vi "order-tracks-test.vi"(1 "Order Settings":T1={"pulses per rev"=1, "trigger level (V)"=2.5, "max order"=64.0, "order resolution"=0.1, "window"=1, "averaging parameters"={"averaging mode"=enum."No averaging", "weighting mode"=enum."Linear", "number of averages"=1, "linear mode"=enum."One shot"}, "order ranges"=[{"start"=0.8, "stop"=1.2}, {"start"=1.8, "stop"=2.2}, {"start"=23.8, "stop"=24.2}]}, 4 "Noise (g rms)":dbl=0.01, 5 "Phases (deg)":dbl[](array[numeric])=[30.0, 0.0, 0.0, 0.0, 0.0], 6 "Orders":dbl[](array[numeric])=[1.0, 2.0, 3.57, 4.0, 24.0], 7 "Amplitudes (g pk)":dbl[](array[numeric])=[0.5, 0.2, 0.1, 0.05, 0.3], 8 "error in (no error)":errorcluster, 9 "Duration (s)":dbl=30.0, 10 "Ramps":T2(array[cluster]), 11 "Base RPM":dbl=3000.0) -> (0 "error out":errorcluster, 2 "True RPM":dbl[](array[numeric]), 3 "Values":dbl[][](array[numeric]))   [LabVIEW 2026]
doc: "Unit-test harness for OrderTracks.vi. Synthesises accel (sum of order sines, peak amplitudes, uniform noise) and a 1 ppr 0-5 V square tach (rising edge at shaft angle 0) for rpm(t) = Base RPM + sum of linear ramps, cuts it into 0.1 s blocks (5120 S @ 51.2 kS/s) and calls OrderTracks.vi block by block like FlexLogger Process.vi does (Data In = [accel, tach], reset? TRUE on block 0). Returns NUMERIC arrays only: Values [blocks x (2 + order ranges)] = RPM, order amplitudes (g rms); True RPM at each block centre."
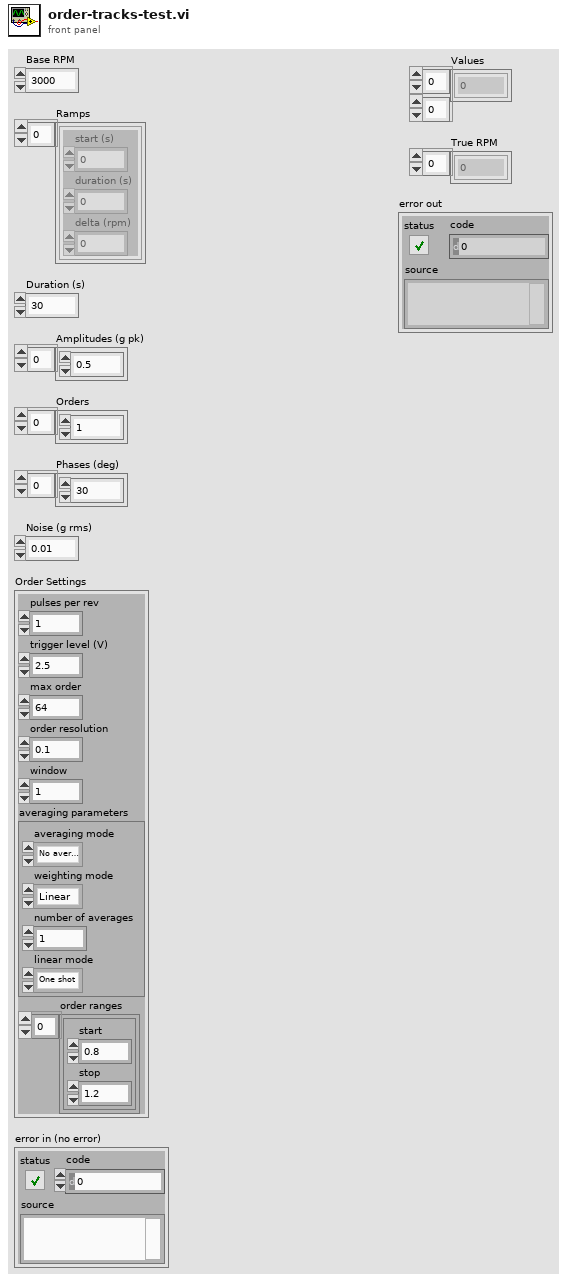
[diagram p1: front panel]
types:
  T1 = cluster{"pulses per rev":i32, "trigger level (V)":dbl, "max order":dbl, "order resolution":dbl, "window":u32, "averaging parameters":cluster{"averaging mode":enum16{"No averaging", "Vector averaging", "RMS averaging", "Peak hold"}, "weighting mode":enum16{"Linear", "Exponential"}, "number of averages":u32, "linear mode":enum16{"One shot", "Auto restart"}}, "order ranges":cluster{"start":dbl, "stop":dbl}[]}
  T2 = cluster{"start (s)":dbl, "duration (s)":dbl, "delta (rpm)":dbl}[]
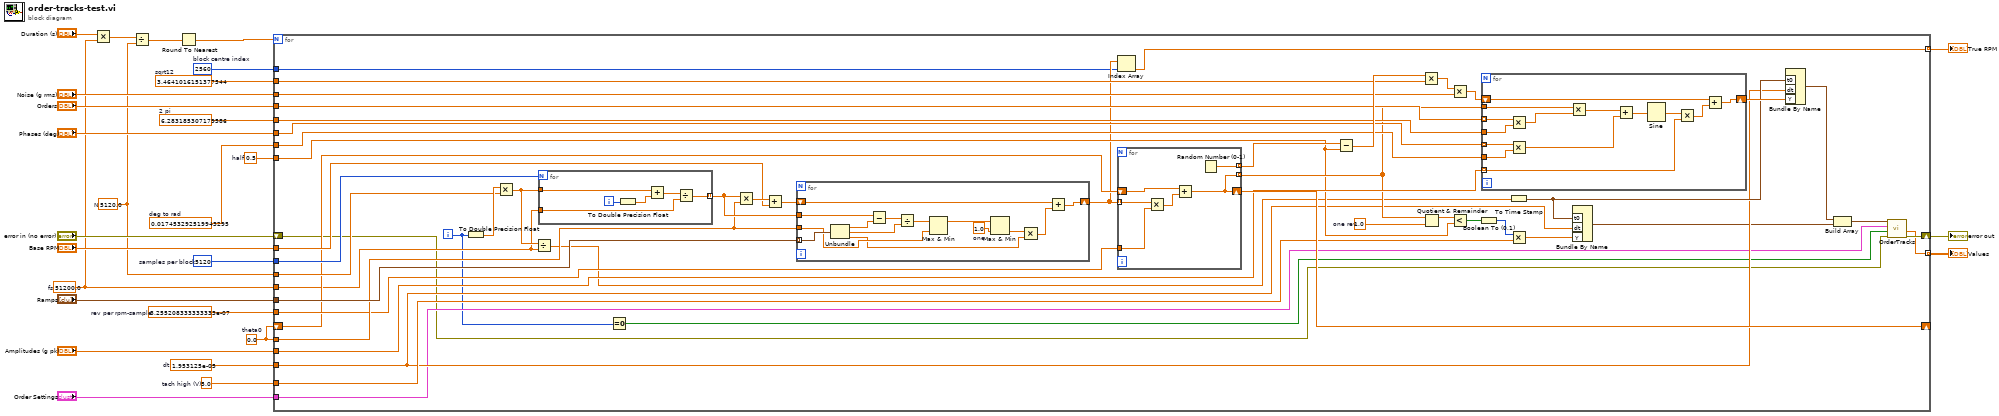
[diagram p0: block diagram]
diagram:
  w6 = 2560  # block centre index
  w7 = 5.0  # tach high (V)
  w8 = 6.283185307179586  # 2 pi
  w9 = 0.017453292519943295  # deg to rad
  w10 = 0.5  # half
  w11 = 3.4641016151377544  # sqrt12
  w12 = 1.953125e-05  # dt
  w13 = 3.255208333333333e-07  # rev per rpm-sample
  w5 = 0.0  # theta0
  w14 = 5120.0  # N
  w15 = 5120  # samples per block
  w16 = 51200.0  # fs
  n1 = Multiply(x="Duration (s)", y=w16) -> (x*y=w26:dbl)
  n2 = Divide(x=w26, y=w14) -> (x/y=w25:dbl)
  n3 = Round To Nearest(number=w25) -> (nearest integer value=w4:dbl)
  n4 = for {
    N: w4 -> [_]
    shift-right: [w66] -> _
    shift-left: w5 -> [w65]
    shift-right: [w33] -> w1
    shift-left: "error in (no error)" -> [w34]
    tunnel: "Base RPM" -> [w72]
    tunnel: "Ramps" -> [w71]
    tunnel: "Amplitudes (g pk)" -> [w58]
    tunnel: "Orders" -> [w59]
    tunnel: "Phases (deg)" -> [w57]
    tunnel: "Noise (g rms)" -> [w60]
    tunnel: "Order Settings" -> [w36]
    tunnel: w16 -> [w45]
    tunnel: w15 -> [w74]
    tunnel: w14 -> [w75]
    tunnel: w13 -> [w67]
    tunnel: w12 -> [w41]
    tunnel: w11 -> [w62]
    tunnel: w10 -> [w50]
    tunnel: w9 -> [w55]
    tunnel: w8 -> [w56]
    tunnel: w7 -> [w47]
    tunnel: w6 -> [w31]
    tunnel: w5 -> [w69]
    tunnel: [w30] -> w3 mode=indexing
    tunnel: [w29] -> w2 mode=indexing
    i -> [w28]
    w52 = 1.0  # one rev
    n5 = To Double Precision Float(number=w28) -> (double precision float=w76:dbl)
    n6 = Multiply(x=w76, y=w75) -> (x*y=w46:dbl)
    n7 = Divide(x=w46, y=w45) -> (x/y=w44:dbl)
    n8 = for {
      N: w74 -> [_]
      tunnel: w46 -> [w116]
      tunnel: w45 -> [w113]
      tunnel: [w112] -> w70 mode=indexing
      i -> [w111]
      n9 = To Double Precision Float(number=w111) -> (double precision float=w115:dbl)
      n10 = Add(x=w116, y=w115) -> (x+y=w114:dbl)
      n11 = Divide(x=w114, y=w113) -> (x/y=w112:dbl)
    }
    n12 = Equal To 0?(x=w28) -> (x = 0?=w35:bool)
    n13 = Multiply(x=w70, y=w69) -> (x*y=w73:dbl[])
    n14 = Add(x=w73, y=w72) -> (x+y=w68:dbl[])
    n15 = for {
      tunnel: w71 -> [w110] mode=indexing
      tunnel: w70 -> [w109]
      tunnel: w69 -> [w104]
      shift-right: [w97] -> w32
      shift-left: w68 -> [w99]
      w102 = 1.0  # one
      n16 = Unbundle(w110) -> ("start (s)"=w108:dbl, "duration (s)"=w106:dbl, "delta (rpm)"=w100:dbl)
      n17 = Subtract(x=w109, y=w108) -> (x-y=w107:dbl[])
      n18 = Divide(x=w107, y=w106) -> (x/y=w105:dbl[])
      n19 = Max & Min(x=w105, y=w104) -> (max(x,y)=w103:dbl[])  [unwired: 1 out]
      n20 = Max & Min(x=w103, y=w102) -> (min(x,y)=w101:dbl[])  [unwired: 1 out]
      n21 = Multiply(x=w101, y=w100) -> (x*y=w98:dbl[])
      n22 = Add(x=w99, y=w98) -> (x+y=w97:dbl[])
    }
    n23 = Index Array(array=w32, index=w31) -> (element=w29:dbl)
    n24 = for {
      tunnel: w32 -> [w96] mode=indexing
      tunnel: w67 -> [w95]
      shift-right: [w92] -> w66
      shift-left: w65 -> [w94]
      tunnel: [w92] -> w53 mode=indexing
      tunnel: [w91] -> w64 mode=indexing
      n25 = Multiply(x=w96, y=w95) -> (x*y=w93:dbl)
      n26 = Add(x=w94, y=w93) -> (x+y=w92:dbl)
      n27 = Random Number (0-1)() -> (number: 0 to 1=w91:dbl)
    }
    n28 = Subtract(x=w64, y=w50) -> (x-y=w63:dbl[])
    n29 = Multiply(x=w63, y=w62) -> (x*y=w61:dbl[])
    n30 = Quotient & Remainder(x=w53, y=w52) -> (x-y*floor(x/y)=w51:dbl[])  [unwired: 1 out]
    n31 = Multiply(x=w61, y=w60) -> (x*y=w54:dbl[])
    n32 = Less?(x=w51, y=w50) -> (x < y?=w49:bool[])
    n33 = Boolean To (0,1)(Boolean=w49) -> (0, 1=w48:i16[])
    n34 = for {
      tunnel: w59 -> [w90] mode=indexing
      tunnel: w58 -> [w80] mode=indexing
      tunnel: w57 -> [w86] mode=indexing
      tunnel: w53 -> [w88]
      tunnel: w56 -> [w89]
      tunnel: w55 -> [w85]
      shift-right: [w77] -> w43
      shift-left: w54 -> [w79]
      n35 = Multiply(x=w90, y=w89) -> (x*y=w87:dbl)
      n36 = Multiply(x=w86, y=w85) -> (x*y=w83:dbl)
      n37 = Multiply(x=w88, y=w87) -> (x*y=w84:dbl[])
      n38 = Add(x=w84, y=w83) -> (x+y=w82:dbl[])
      n39 = Sine(x=w82) -> (sin(x)=w81:dbl[])
      n40 = Multiply(x=w81, y=w80) -> (x*y=w78:dbl[])
      n41 = Add(x=w79, y=w78) -> (x+y=w77:dbl[])
    }
    n42 = Multiply(x=w48, y=w47) -> (x*y=w40:dbl[])
    n43 = To Time Stamp(1:w44) -> (0:w42:timestamp)
    n44 = Bundle By Name("t0"=w42, "dt"=w41, "Y"=w40) -> (w38:waveform(dbl))  [unwired: 1 in]
    n45 = Bundle By Name("t0"=w42, "dt"=w41, "Y"=w43) -> (w39:waveform(dbl))  [unwired: 1 in]
    n46 = Build Array(w39, w38) -> (w37:waveform(dbl)[])
    n47 = call "OrderTracks.vi"("error in (no error)"=w34, "reset? (F)"=w35, "Order Settings"=w36, "Data In"=w37) -> ("error out"=w33:errorcluster, "Values"=w30:dbl[])  [unwired: 5 in, 1 out]
  }
  "Values" <- w3
  "True RPM" <- w2
  "error out" <- w1
